vi "Config_Resolve_Plugins.vi"(8 "error in (no error)":errorcluster={"status"=FALSE, "code"=0, "source"="\"\""}, 10 "deployment index":string, 11 "Manifest list":string) -> (0 "error out":errorcluster={"status"=FALSE, "code"=0, "source"="\"\""}, 2 "status ok":bool, 3 "Resolved plugin registry":string)   [LabVIEW 2026]
doc: "INTENT: Check plugin package availability. LOGIC: Match plugin ID/version, target, connector signature and resource permissions."
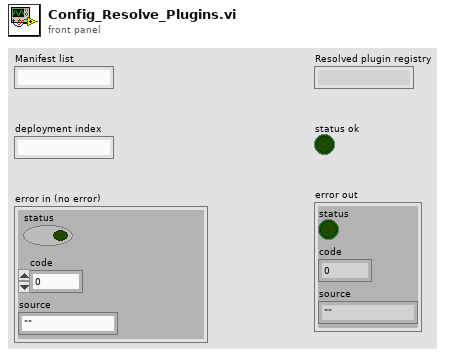
[diagram p1: front panel]
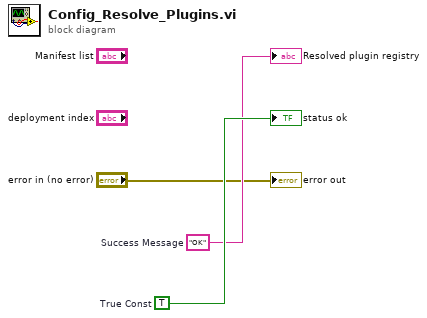
[diagram p0: block diagram]
diagram:
  w3 = TRUE  # True Const
  w2 = "OK"  # Success Message
  "Resolved plugin registry" <- w2
  "status ok" <- w3
  "error out" <- "error in (no error)"
